vi "Convert Boolean Output Value to Register.vi"(8 "error in (no error)":errorcluster, 10 "Boolean Output in":T1, 11 "Plugin in":refnum<class "Modbus.lvclass">) -> (0 "error out":errorcluster, 1 "Value":bool, 2 "Boolean Output out":T1, 3 "Plugin out":refnum<class "Modbus.lvclass">, 4 "Data Valid":bool)   [LabVIEW 2026, in "Modbus.lvlib" / "Modbus.lvclass"]
uses:
  Modbus.lvclass
  Types/Boolean Data.ctl
  Types/Modbus Table.ctl
  C:/Program Files/National Instruments/LabVIEW 2026/vi.lib/FlexLogger/SDK/PluginSDK.lvlibp/PEFClasses/SDK/Plugin/Plugin.lvclass
  <vilib>/FlexLogger/SDK/PluginSDK.lvlibp/PEFClasses/SDK/Plugin/Plugin.lvclass
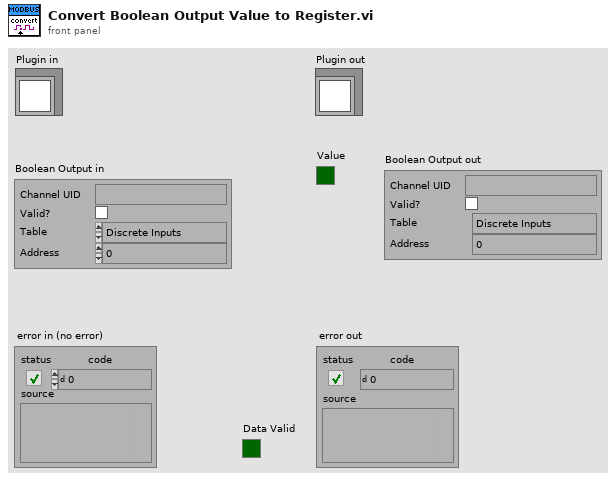
[diagram p1: front panel]
types:
  T1 = typedef "Modbus.lvlib/Modbus.lvclass/Boolean Data.ctl" = cluster{"Channel UID":string, "Valid?":bool, "Table":T2, "Address":i32}
  T2 = typedef "Modbus.lvlib/Modbus.lvclass/Modbus Table.ctl" = enum16{"Discrete Inputs", "Coils", "Input Registers", "Holding Registers"}
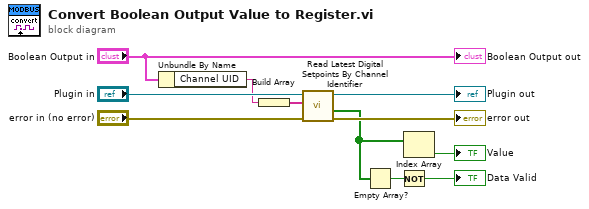
[diagram p0: block diagram]
diagram:
  n1 = Unbundle By Name("Boolean Output in") -> ("Channel UID"=w8:string)
  n2 = Build Array(w8) -> (w9:string[])
  n3 = call <vilib>:"Read Latest Digital Setpoints By Channel Identifier.vi"("error in (no error)"="error in (no error)", "Unique Channel Identifiers (empty = all)"=w9, "Plugin in"="Plugin in") -> ("error out"=→"error out":errorcluster, "Values"=w5:bool[], "Plugin out"=→"Plugin out":refnum<class "Modbus.lvclass">)  [unwired: 5 in, 1 out]
  n4 = Empty Array?(array=w5) -> (empty?=w4:bool)
  n5 = Not(x=w4) -> (.not. x?=→"Data Valid":bool)
  n6 = Index Array(array=w5) -> (element=→"Value":bool)  [unwired: 1 in]
  "Boolean Output out" <- "Boolean Output in"
